vi "Biorreactor.vi"() -> ()   [LabVIEW 2013]
uses:
  data.ctl
  event.ctl
  <vilib>/DAQmx/create/channels.llb/DAQmx Create Channel (AO-Voltage-Basic).vi
  <vilib>/DAQmx/create/channels.llb/DAQmx Create Channel (AI-Voltage-Basic).vi
  <vilib>/DAQmx/write.llb/DAQmx Write (Analog 1D DBL NChan 1Samp).vi
  <vilib>/DAQmx/read.llb/DAQmx Read (Analog 1D DBL NChan 1Samp).vi
panel:
  in  "Activación":bool
  in  "Activación":bool
  in  "Bomba 2":bool
  in  "Bomba 1":bool
  in  "manual":bool=TRUE
  in  "Umbral control B 2":dbl=7.0 format="%#_13g"
  in  "Umbral control B 1":dbl=7.0 format="%#_13g"
  in  "bOD2":dbl=1.2462 format="%#_13g"
  in  "a2OD2":dbl=0.5407 format="%#_13g"
  out "Volt OD 2 (V4)":dbl format="%#_2g"
  out "Volt PH 2 (V3)":dbl format="%#_2g"
  out "OD 2":dbl(graph)
  out "PH 2":dbl(graph)
  in  "bpH2":dbl=1.2462 format="%#_13g"
  in  "apH2":dbl=0.5407 format="%#_13g"
  out "OD 2 [%]":dbl(slide) scale=0.0..100.0
  out "pH 2":dbl(slide) scale=0.0..20.0
  out "periodo en milisegundos":dbl
  in  "periodo muestreo (Seg.)":dbl=1.0 format="%#_13g"
  out "Tiempo transcurrido":dbl
  in  "Stop Button":bool
  in  "Play Button":bool
  in  "bOD1":dbl=1.2462 format="%#_13g"
  in  "aOD1":dbl=0.5407 format="%#_13g"
  out "Volt OD 1 (V2)":dbl format="%#_2g"
  out "Volt PH 1 (V1)":dbl format="%#_2g"
  in  "Save Data":bool
  in  "Record":bool
  out "OD 1":dbl(graph)
  out "PH 1":dbl(graph)
  in  "bpH1":dbl=1.2462 format="%#_13g"
  in  "apH1":dbl=0.5407 format="%#_13g"
  out "OD 1 [%]":dbl(slide) scale=0.0..100.0
  out "pH 1":dbl(slide) scale=0.0..20.0
  in  "exit":bool
  # "Guardado de datos"
  # "Calibración pH"
  # "Calibración pH"
  # "pH=apH1*V3+bpH1"
  # "pH=apH1*V1+bpH1"
  # "Calibración OD"
  # "Calibración OD"
  # "OD=aOD2*V4+bOD2"
  # "OD=aOD1*V2+bOD1"
  # "Desarrollado por Cristian Castro Lagos - Laboratorio de Control  - EIE PUCV"
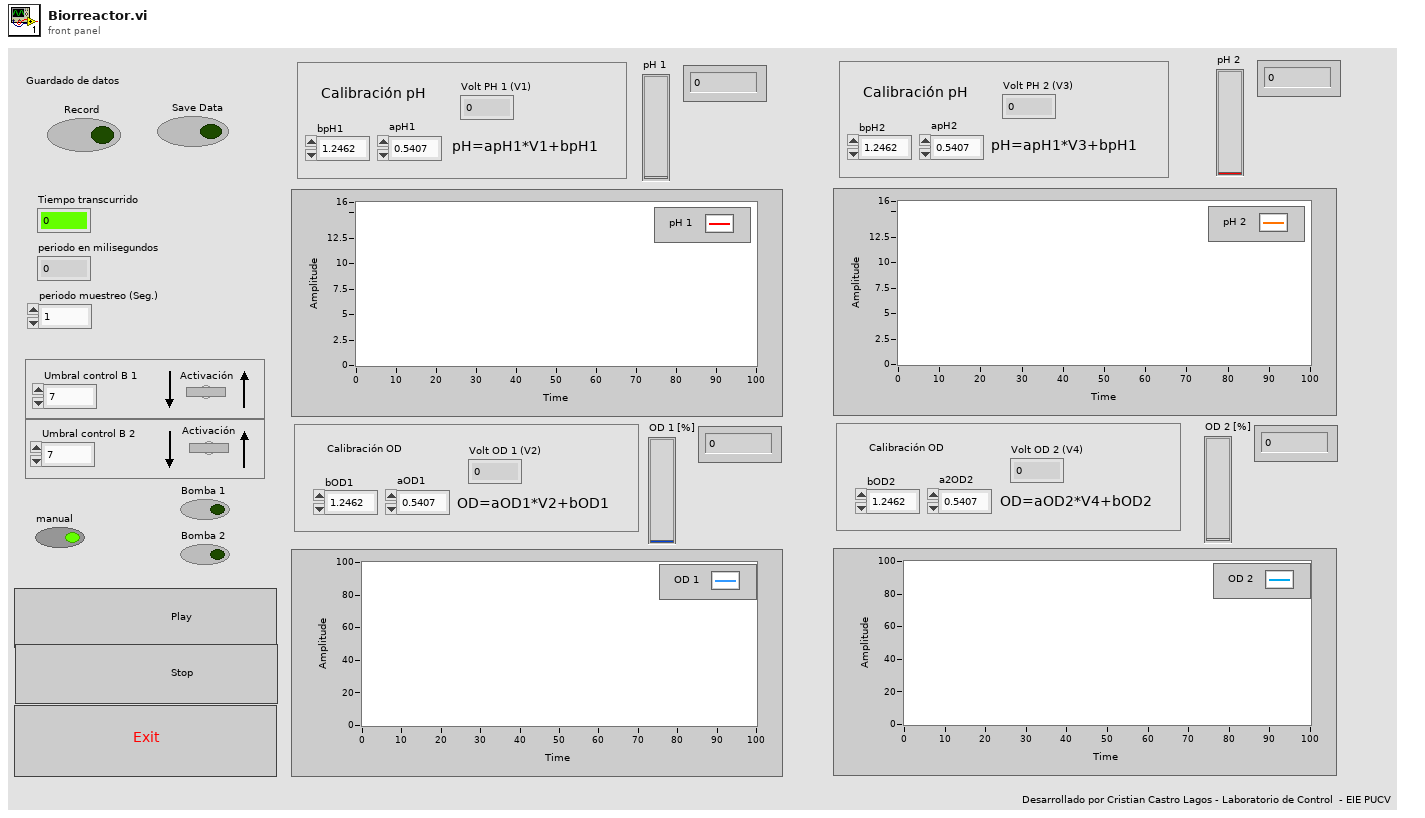
[diagram p1: front panel]
types:
  T1 = typedef "event.ctl" = enum16{"initialize", "run", "stop", "exit"}
  T2 = typedef "data.ctl" = cluster{"PH 1":dbl, "t":dbl, "OD 1":dbl, "OD 2":dbl, "PH 2":dbl}
  T3 = enum32{"invalid app kind", "Development System", "Run Time System", "Student Edition", "Embedded LabVIEW", "Evaluation", "Custom"}
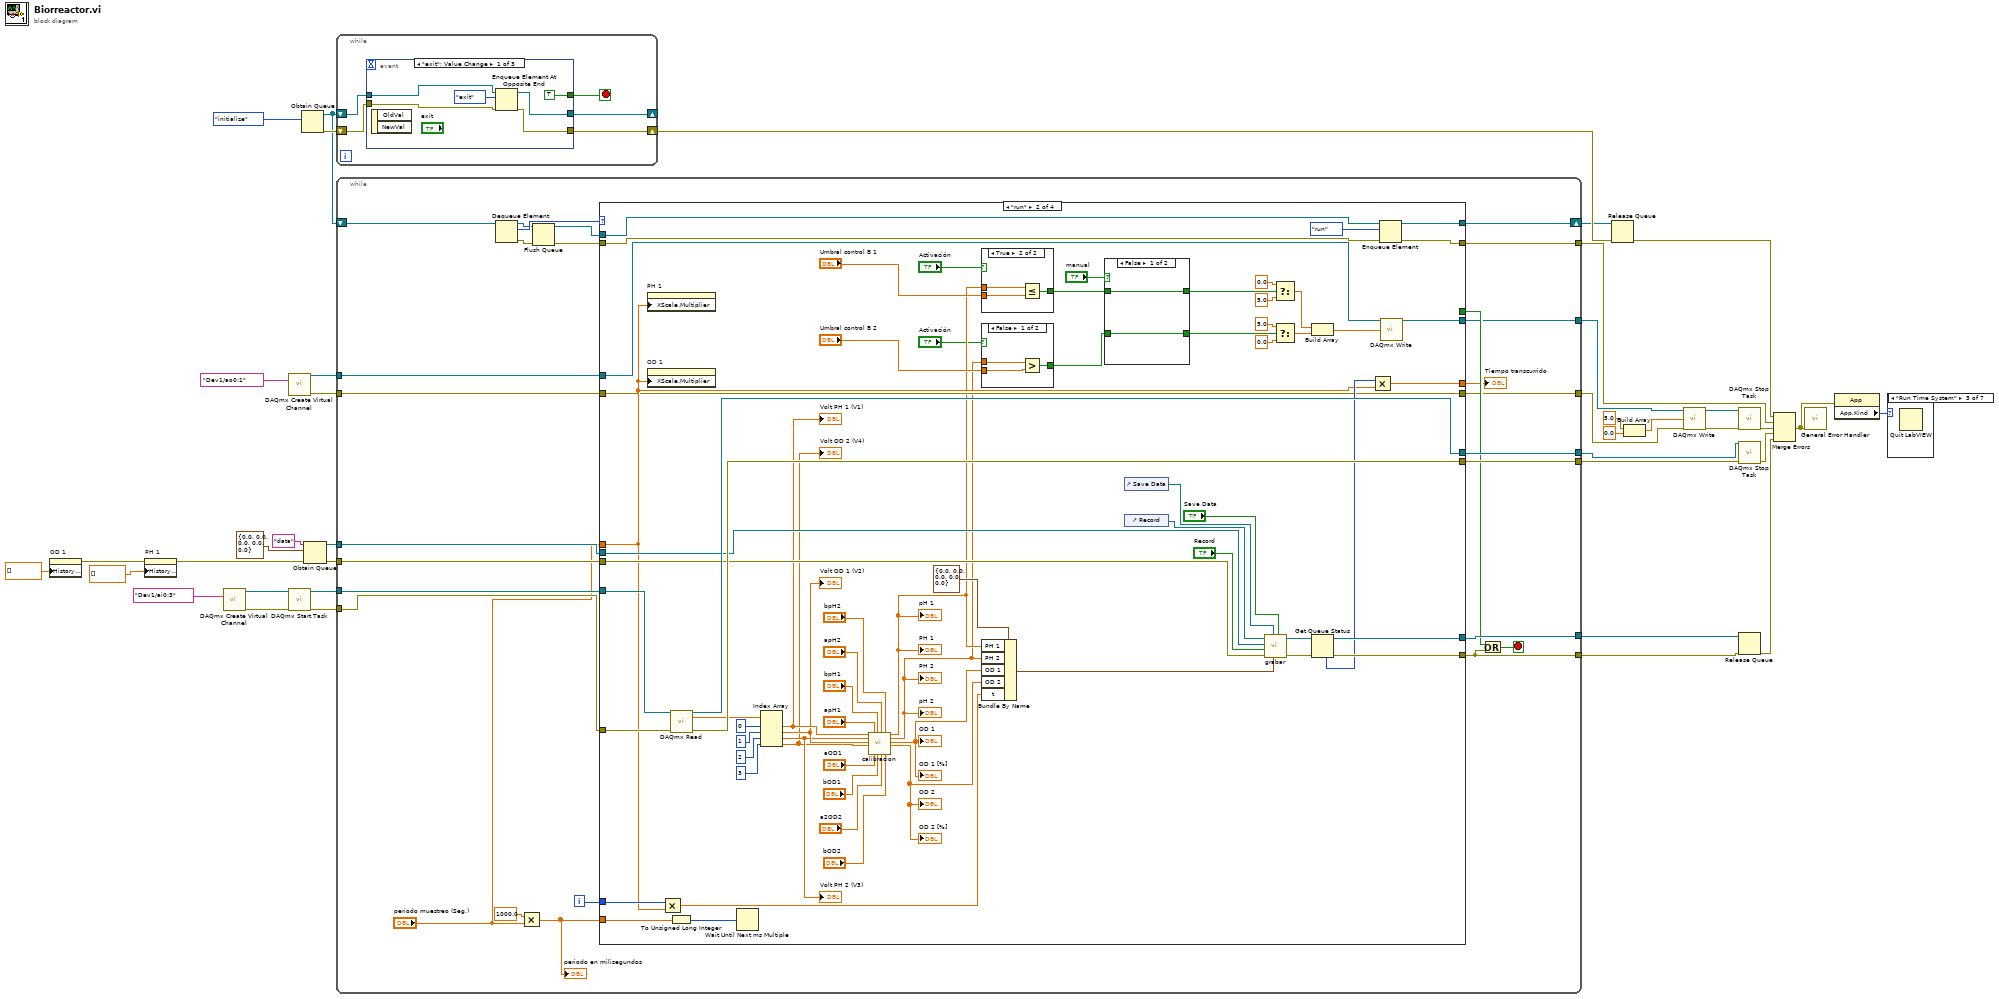
[diagram p0: block diagram]
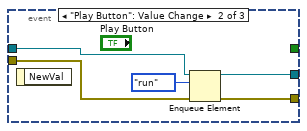
[diagram p8: hidden frame]
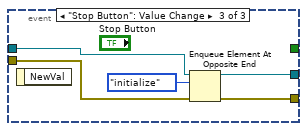
[diagram p9: hidden frame]
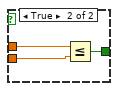
[diagram p11: hidden frame]
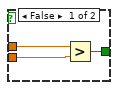
[diagram p12: hidden frame]
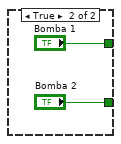
[diagram p13: hidden frame]
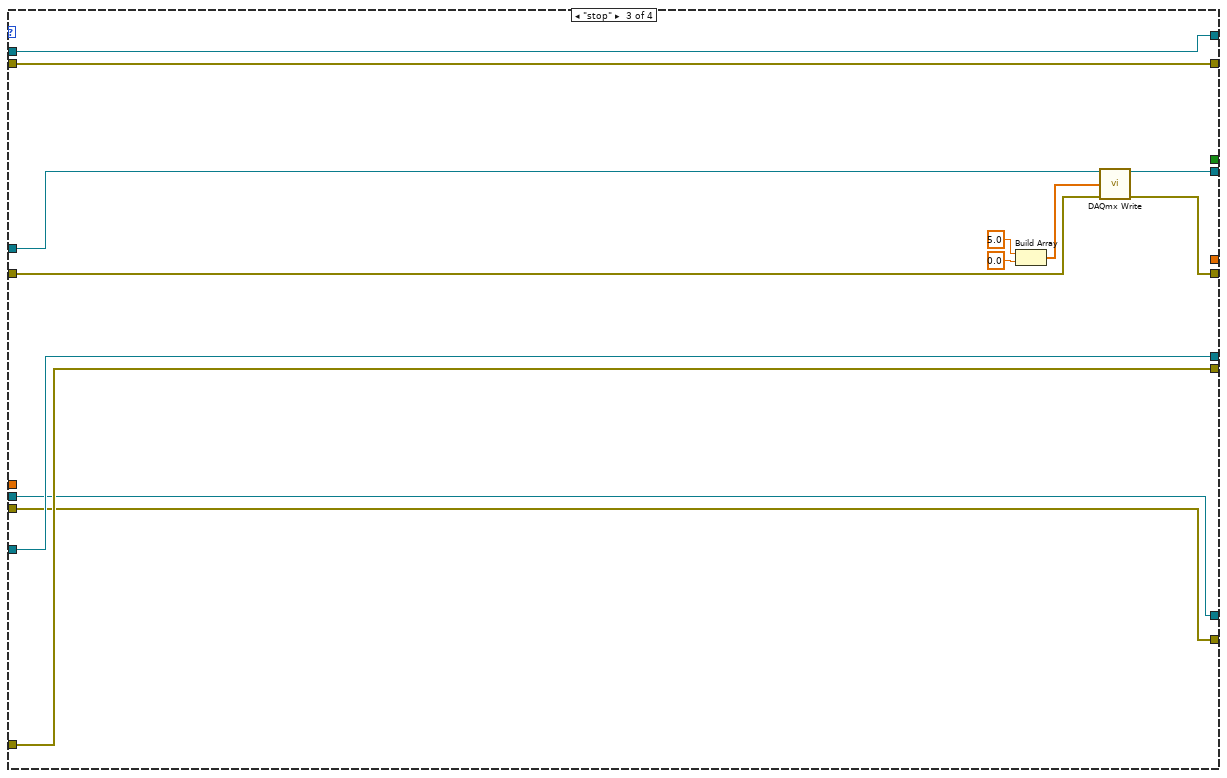
[diagram p14: hidden frame]
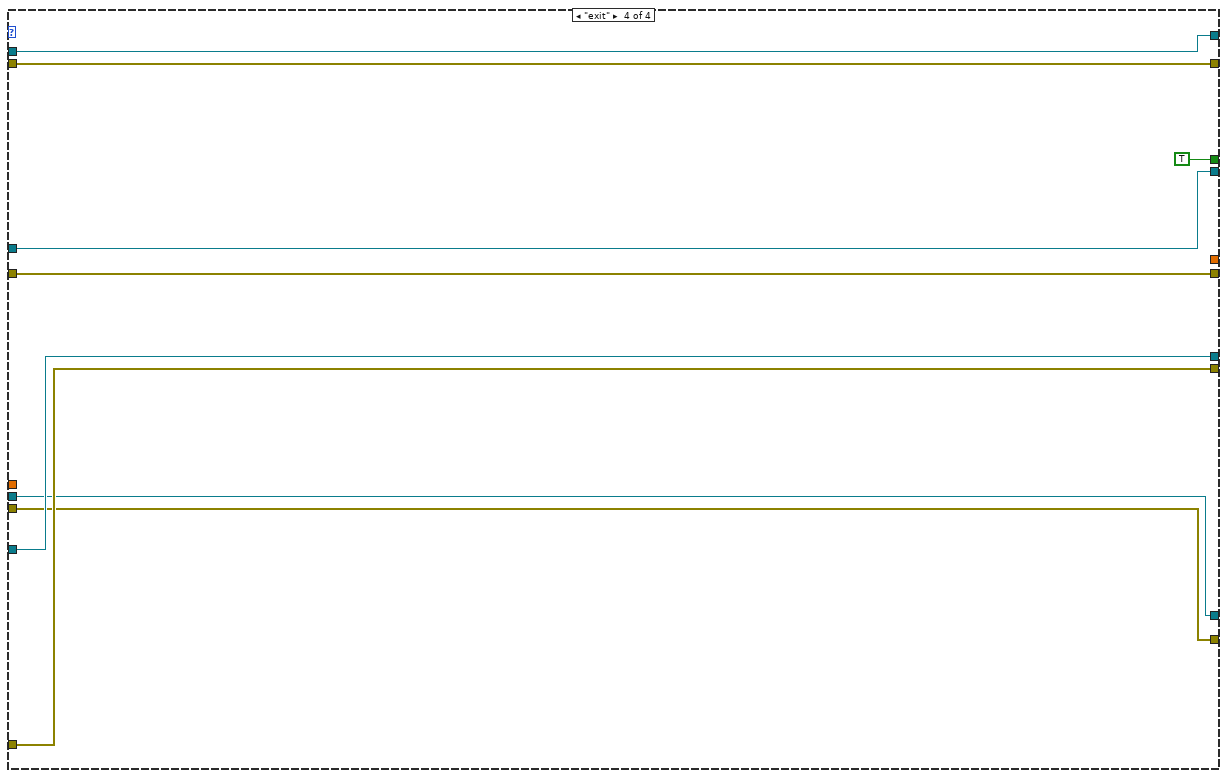
[diagram p15: hidden frame]
diagram:
  n1 = property on="OD 1" class="WFChart (strict)"("History Data"=dbl[] []) -> (error out=w26:errorcluster)  [unwired: 2 in, 1 out]
  n2 = property on="PH 1" class="WFChart (strict)"(error in=w26, "History Data"=dbl[] []) -> (error out=w27:errorcluster)  [unwired: 1 in, 1 out]
  n3 = call-poly <vilib>:"DAQmx Create Virtual Channel.vi"("physical channels"=tag "Dev1/ai0:3") -> ("task out"=w3:refnum<k21>, "error out"=w2:errorcluster)  [unwired: 13 in]
  n4 = call-poly <vilib>:"DAQmx Create Virtual Channel.vi"("physical channels"=tag "Dev1/ao0:1") -> ("task out"=w16:refnum<k21>, "error out"=w15:errorcluster)  [unwired: 13 in]
  n5 = call <vilib>:"DAQmx Start Task.vi"("task/channels in"=w3, "error in"=w2) -> ("task out"=w39:refnum<k21>, "error out"=w36:errorcluster)  [unwired: 12 in]
  n6 = Obtain Queue(element data type=event."initialize") -> (queue out=w20:refnum<queue>, error out=w23:errorcluster)  [unwired: 4 in, 1 out]
  n7 = Obtain Queue(name (unnamed)="data", element data type=T2 {"PH 1"=0.0, "t"=0.0, "OD 1"=0.0, "OD 2"=0.0, "PH 2"=0.0} ("output cluster"), error in (no error)=w27) -> (queue out=w31:refnum<queue>, error out=w32:errorcluster)  [unwired: 2 in, 1 out]
  n8 = while {
    shift-right: [w44] -> _
    shift-left: w20 -> [w43]
    shift-right: [w41] -> w22
    shift-left: w23 -> [w42]
    stop <- w40 stop-if-true
    n9 = event shown="[0] \"exit\": Value Change" {
      selector: _ -> [_ _ _]
      dyn-events: _ -> [_ _ _]
      timeout: _ -> [_ _ _]
      tunnel: [w47 w52 w57] -> w44
      tunnel: w43 -> [w48 w53 w58]
      tunnel: w42 -> [w50 w55 w60]
      tunnel: [w49 w54 w59] -> w41
      tunnel: [TRUE _ _] -> w40
      event "exit": Value Change {
        n10 = event-data() -> ()  [unwired: 1 in, 2 out]
        n11 = Enqueue Element At Opposite End(queue=w48, element=event."exit", error in (no error)=w50) -> (queue out=w47:refnum<queue>, error out=w49:errorcluster)  [unwired: 1 in, 1 out]
      }
      event "Play Button": Value Change {
        n12 = event-data() -> ()  [unwired: 1 in, 1 out]
        n13 = Enqueue Element(queue=w53, element=event."run", error in (no error)=w55) -> (queue out=w52:refnum<queue>, error out=w54:errorcluster)  [unwired: 1 in, 1 out]
      }
      event "Stop Button": Value Change {
        n14 = event-data() -> ()  [unwired: 1 in, 1 out]
        n15 = Enqueue Element At Opposite End(queue=w58, element=event."initialize", error in (no error)=w60) -> (queue out=w57:refnum<queue>, error out=w59:errorcluster)  [unwired: 1 in, 1 out]
      }
    }
  }
  n16 = while {
    tunnel: w39 -> [w87]
    tunnel: [w86] -> w38
    tunnel: [w85] -> w37
    tunnel: w36 -> [w84]
    tunnel: [w83] -> w34
    tunnel: [w77] -> w33
    tunnel: w32 -> [w82]
    tunnel: w31 -> [w81]
    shift-right: [w74] -> w17
    shift-left: w20 -> [w79]
    tunnel: [w72] -> w19
    tunnel: w16 -> [w64]
    tunnel: [w63] -> w10
    tunnel: [w61] -> w8
    tunnel: w15 -> [w62]
    i -> [w80]
    stop <- w75 stop-if-true
    n17 = Dequeue Element(queue=w79) -> (queue out=w70:refnum<queue>, element=w78:T1, error out=w73:errorcluster)  [unwired: 2 in, 1 out]
    n18 = Multiply(x=1000.0, y="periodo muestreo (Seg.)") -> (x*y=w67:dbl)
    "periodo en milisegundos" <- w67
    n19 = Flush Queue(queue=w70, error in (no error)=w73) -> (queue out=w69:refnum<queue>, error out=w71:errorcluster)  [unwired: 1 out]
    n20 = case shown="\"run\"" w78 {
      tunnel: w87 -> [w93 w163 w192 w201]
      tunnel: [w93 w162 w192 w201] -> w86
      tunnel: [w92 w161 w191 w200] -> w85
      tunnel: w84 -> [w92 w160 w191 w200]
      tunnel: [_ w135 _ _] -> w65
      tunnel: [w95 w156 w190 w199] -> w83
      tunnel: w82 -> [w94 w155 w189 w198]
      tunnel: w81 -> [w95 w154 w190 w199]
      tunnel: w80 -> [_ w153 _ _]
      tunnel: [w94 w149 w189 w198] -> w77
      tunnel: [_ _ _ TRUE] -> w76
      tunnel: w69 -> [w91 w143 w188 w196]
      tunnel: [w91 w142 w188 w196] -> w74
      tunnel: w71 -> [w90 w141 w187 w195]
      tunnel: [w90 w140 w187 w195] -> w72
      tunnel: w67 -> [_ w139 _ _]
      tunnel: "periodo muestreo (Seg.)" -> [_ w136 _ _]
      tunnel: w64 -> [w89 w98 w185 w194]
      tunnel: [w89 w134 w184 w194] -> w63
      tunnel: w62 -> [w88 w133 w181 w193]
      tunnel: [w88 w133 w180 w193] -> w61
      frame "initialize", Default {
      }
      frame "run" {
        n21 = property on="PH 1" class="WFChart (strict)"("XScale.Multiplier"=w136) -> ()  [unwired: 2 in, 2 out]
        n22 = property on="OD 1" class="WFChart (strict)"("XScale.Multiplier"=w136) -> ()  [unwired: 2 in, 2 out]
        n23 = Multiply(x=w153, y=w136) -> (x*y=w108:dbl)
        n24 = call-poly <vilib>:"DAQmx Read.vi"("task/channels in"=w163, "error in"=w160) -> ("task out"=w162:refnum<k21>, "data"=w148:dbl[], "error out"=w161:errorcluster)  [unwired: 11 in]
        n25 = To Unsigned Long Integer(number=w139) -> (unsigned 32bit integer=w138:u32)
        n26 = Wait Until Next ms Multiple(millisecond multiple=w138) -> ()  [unwired: 1 out]
        n27 = Index Array(array=w148, index #1=0 ("index"), index #2=1 ("index"), index #3=2 ("index"), index #4=3 ("index")) -> (element #1=w128:dbl, element #2=w127:dbl, element #3=w126:dbl, element #4=w125:dbl)
        "Volt PH 1 (V1)" <- w128
        "Volt OD 1 (V2)" <- w127
        "Volt PH 2 (V3)" <- w126
        "Volt OD 2 (V4)" <- w125
        n28 = call "calibracion.vi"("voltaje PH 1"=w128, "voltaje PH 2"=w126, "Voltaje OD 1"=w127, "Voltaje OD 2"=w125, "aPh1"="apH1", "aOD1"="aOD1", "bPh1"="bpH1", "bOD1"="bOD1", "aPh2"="apH2", "aOD2"="a2OD2", "bPh2"="bpH2", "bOD2"="bOD2") -> ("PH 1"=w107:dbl, "PH 2"=w106:dbl, "OD 1"=w105:dbl, "OD 2"=w104:dbl)  [unwired: 4 in]
        "PH 1" <- w107
        "OD 1" <- w105
        "pH 1" <- w107
        "OD 1 [%]" <- w105
        "OD 2" <- w104
        "pH 2" <- w106
        "OD 2 [%]" <- w104
        "PH 2" <- w106
        n29 = case shown="True" "Activación" {
          tunnel: "Umbral control B 1" -> [w170 w175]
          tunnel: w107 -> [w171 w174]
          tunnel: [w172 w173] -> w102
          frame False {
            n30 = Greater?(x=w171, y=w170) -> (0:w172:bool)
          }
          frame True {
            n31 = Less Or Equal?(x=w174, y=w175) -> (x <= y?=w173:bool)
          }
        }
        n32 = case shown="False" "Activación" {
          tunnel: "Umbral control B 2" -> [w164 w169]
          tunnel: w106 -> [w165 w168]
          tunnel: [w166 w167] -> w100
          frame False {
            n33 = Greater?(x=w165, y=w164) -> (0:w166:bool)
          }
          frame True {
            n34 = Less Or Equal?(x=w168, y=w169) -> (x <= y?=w167:bool)
          }
        }
        n35 = Bundle By Name(cluster=T2 {"PH 1"=0.0, "t"=0.0, "OD 1"=0.0, "OD 2"=0.0, "PH 2"=0.0} ("output cluster"), "PH 1"=w107, "PH 2"=w106, "OD 1"=w105, "OD 2"=w104, "t"=w108) -> (w151:T2)
        n36 = case shown="False" "manual" {
          tunnel: w102 -> [w177 _]
          tunnel: [w177 "Bomba 1"] -> w101
          tunnel: w100 -> [w176 _]
          tunnel: [w176 "Bomba 2"] -> w99
          frame False {
          }
          frame True {
          }
        }
        n37 = control-ref of="Save Data"() -> (w144:refnum<vi>)
        n38 = control-ref of="Record"() -> (w145:refnum<vi>)
        n39 = call "grabar.vi"("Save Data"="Save Data", "output cluster"=w151, "Bool Refnum in"=w144, "error in (no error)"=w155, "Record"="Record", "queue in"=w154, "Boolean in"=w145) -> ("error out"=w150:errorcluster, "Queue out"=w157:refnum<queue>)  [unwired: 3 in]
        n40 = Select(t=0.0, s=w101, f=5.0) -> (s? t:f=w113:dbl)
        n41 = Select(t=5.0, s=w99, f=0.0) -> (s? t:f=w110:dbl)
        n42 = Build Array(w113, w110) -> (w132:dbl[])
        n43 = Get Queue Status(queue=w157, error in (no error)=w150) -> (queue out=w156:refnum<queue>, error out=w149:errorcluster, # elements in queue=w137:i32)  [unwired: 1 in, 5 out]
        n44 = Multiply(x=w137, y=w136) -> (x*y=w135:dbl)
        n45 = Enqueue Element(queue=w143, element=event."run" ("f"), error in (no error)=w141) -> (queue out=w142:refnum<queue>, error out=w140:errorcluster)  [unwired: 1 in, 1 out]
        n46 = call-poly <vilib>:"DAQmx Write.vi"("task/channels in"=w98, "data"=w132) -> ("task out"=w134:refnum<k21>)  [unwired: 11 in, 2 out]
      }
      frame "stop" {
        n47 = Build Array(5.0 ("element"), 0.0 ("f")) -> (w186:dbl[])
        n48 = call-poly <vilib>:"DAQmx Write.vi"("task/channels in"=w185, "data"=w186, "error in"=w181) -> ("task out"=w184:refnum<k21>, "error out"=w180:errorcluster)  [unwired: 10 in, 1 out]
      }
      frame "exit" {
      }
    }
    "Tiempo transcurrido" <- w65
    n49 = Or(x=w76, y=w77) -> (x .or. y?=w75:bool)
  }
  n50 = Release Queue(queue=w17, error in (no error)=w22) -> (error out=w18:errorcluster)  [unwired: 1 in, 2 out]
  n51 = Build Array(5.0 ("Motor 3"), 0.0 ("Motor 4")) -> (w13:dbl[])
  n52 = call-poly <vilib>:"DAQmx Write.vi"("task/channels in"=w10, "data"=w13, "error in"=w8) -> ("task out"=w9:refnum<k21>, "error out"=w7:errorcluster)  [unwired: 10 in, 1 out]
  n53 = call <vilib>:"DAQmx Stop Task.vi"("task/channels in"=w9, "error in"=w7) -> ("error out"=w6:errorcluster)  [unwired: 12 in, 1 out]
  n54 = call <vilib>:"DAQmx Stop Task.vi"("task/channels in"=w38, "error in"=w37) -> ("error out"=w25:errorcluster)  [unwired: 12 in, 1 out]
  n55 = Release Queue(queue=w34, error in (no error)=w33) -> (error out=w24:errorcluster)  [unwired: 1 in, 2 out]
  n56 = Merge Errors(w18, w19, w6, w25, w24) -> (w5:errorcluster)
  n57 = call <vilib>:"General Error Handler.vi"("error in (no error)"=w5) -> ()  [unwired: 10 in, 5 out]
  n58 = property class="App"(error in=w5) -> ("App.Kind"=w4:T3)  [unwired: 1 in, 2 out]
  n59 = case shown="\"Run Time System\"" w4 {
    frame "invalid app kind", Default {
    }
    frame "Development System" {
    }
    frame "Run Time System" {
      n60 = Quit LabVIEW() -> ()  [unwired: 1 in]
    }
    frame "Student Edition" {
    }
    frame "Embedded LabVIEW" {
    }
    frame "Evaluation" {
    }
    frame "Custom" {
    }
  }
